vi "Radar_Schritt.vi"(10 "StateIn":dbl[](array[numeric])=[0.0, 0.0, 0.0, 0.0, 0.0, 0.0, 0.0, 0.0, 0.0, 0.0, 0.0, 0.0, 0.0, 0.0, 0.0, 0.0, 0.0, 0.0, 0.0, 0.0], 11 "Parameters":dbl[](array[numeric])=[0.05, 1.5, 0.0, 1.0, 0.0, 0.0, 0.0, 0.0, 0.0, 0.0, 0.0, 4.0, 20.0, 0.0, 0.0, 0.0, 0.0, 0.0, 0.0, 0.0]) -> (2 "Values":dbl[](array[numeric]), 3 "StateOut":dbl[](array[numeric]))   [LabVIEW 2026]
doc: "AT1B virtual sensor workbench: deterministic model step. Explicit state, no hardware access. See model contract and assumptions."
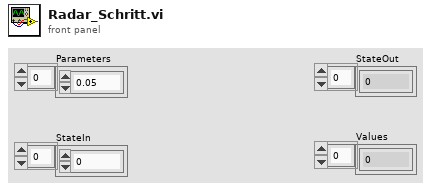
[diagram p1: front panel]
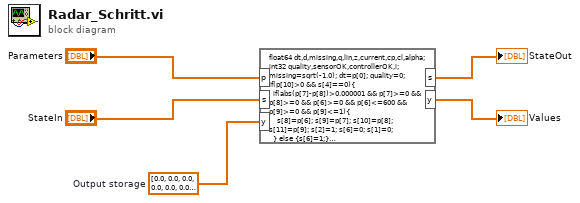
[diagram p0: block diagram]
diagram:
  w3 = dbl[] [0.0, 0.0, 0.0, 0.0, 0.0, 0.0, 0.0, 0.0, 0.0, 0.0, 0.0, 0.0]  # Output storage
  n1 = formula code="float64 dt,d,missing,q,lin,z,current,cp,cl,alpha;\nint32 quality,sensorOK,controllerOK,i;\nmissing=sqrt(-1.0); dt=p[0]; quality=0;\nif(p[10]>0 && s[4]==0){\n  if(abs(p[7]-p[8])>0.000001 && p[7]>=0 && p[8]>=0 && p[6]>=0 && p[6]<=600 && p[9]>=0 && p[9]<=1){\n    s[8]=p[6]; s[9]=p[7]; s[10]=p[8]; s[11]=p[9]; s[2]=1; s[6]=0; s[1]=0;\n  } else {s[6]=1;}\n}\nif(p[19]>0 && s[5]==0){\n  if(p[12]>p[11] && p[11]>=0 && p[12]<=30 && p[13]>=0 && p[13]<=1 && abs(p[15]-p[14])>0.000001 && p[16]>=0 && p[17]<=100 && p[17]>=p[16] && p[18]>=0 && p[18]<=2){\n    for(i=0;i<8;i++){s[12+i]=p[11+i];} s[3]=1; s[6]=0;\n  } else {s[6]=2;}\n}\ns[4]=(p[10]>0); s[5]=(p[19]>0);\nif(s[2]==0){quality=1;} if(s[2]>0 && s[3]==0){quality=2;}\nif(p[3]==0){quality=3;} if(p[4]==0){quality=4;}\nif(dt<=0 || dt>0.25 || p[1]<=0 || p[2]<0 || p[2]>p[1] || abs(p[5])>0.1){quality=9;}\nfor(i=0;i<8;i++){y[i]=missing;} y[8]=0;\nif(quality!=9){s[7]=s[7]+dt;}\nsensorOK=(s[2]>0 && p[3]>0 && p[4]>0 && quality!=9);\nif(sensorOK){\n  d=p[1]-p[2]+p[5];\n  if(s[1]==0){s[0]=d; s[1]=1;} else {alpha=1; if(s[8]>0){alpha=1-exp(-dt/s[8]);} s[0]=s[0]+alpha*(d-s[0]);}\n  q=(s[0]-s[9])/(s[10]-s[9]); if(q<0){q=0;} if(q>1){q=1;} lin=q;\n  if(s[11]>0){z=1-2*q; lin=(acos(z)-z*sqrt(1-z*z))/3.141592653589793;}\n  current=4+16*lin; y[0]=s[0]; y[1]=100*q; y[2]=100*lin; y[3]=current; y[7]=p[2];\n  if(s[3]>0){\n    cp=(current-s[12])/(s[13]-s[12]); if(cp<0){cp=0;} if(cp>1){cp=1;} cl=cp;\n    if(s[14]>0){z=1-2*cp; cl=(acos(z)-z*sqrt(1-z*z))/3.141592653589793;}\n    y[4]=100*cp; y[5]=100*cl; y[6]=s[15]+cl*(s[16]-s[15]);\n    if(s[19]==1){y[8]=(100*cl>=s[17] && 100*cl<=s[18]);}\n    if(s[19]==2){y[8]=(100*cl<s[17] || 100*cl>s[18]);}\n  }\n} else {s[1]=0;}\ny[9]=quality; y[10]=s[6]; y[11]=s[7];"("p"="Parameters", "s"="StateIn", "y"=w3) -> ("s"=→"StateOut":dbl[], "y"=→"Values":dbl[])
